vi "Read current vs temperature_3ch_2.1.1.vi"(8 "stop":bool) -> (0 "X3":cluster{"Y":dbl[], "Y":dbl[]}[](graph), 1 "Zx 4":cluster{"Y":dbl[], "Y":dbl[]}[](graph), 2 "Zx 3":cluster{"Y":dbl[], "Y":dbl[]}[](graph), 3 "Temp vs Time":cluster{"Y":dbl[], "Y":dbl[]}[](graph), 4 "i X":cluster{"Y":dbl[], "Y":dbl[]}[](graph), 5 "X 2":cluster{"Y":dbl[], "Y":dbl[]}[](graph))   [LabVIEW 2013]
uses:
  PPMS_remote/branches/sim-JL/Simulate.glb.vi
  lockin/branches/PPMS-demomode-JL/Lock-in Globles.vi
  SubVI/ITX_Global.vi
panel:
  in  "Tab Control":T1(tab)
  in  "Lockins":u16[](array[ring]) items=["Lock-in #1", "Lock-in #2", "Lock-in #3", "Lock-in #4"]
  out "OSC Configuration":T2(array[cluster])=[{"Signal Type"=enum."Sine Wave", "DC"=0.0005, "Amplitude"=0.001, "frequency"=1.346, "Phase"=0.0}, {"Signal Type"=enum."Sine Wave", "DC"=0.0, "Amplitude"=0.0, "frequency"=1.346, "Phase"=0.0}, {"Signal Type"=enum."Sine Wave", "DC"=0.0, "Amplitude"=0.0, "frequency"=1.346, "Phase"=0.0}, {"Signal Type"=enum."Sine Wave", "DC"=0.0, "Amplitude"=0.0, "frequency"=1.346, "Phase"=0.0}] {"frequency" format="%0.2p"; "Amplitude" format="%0.2p"; "DC" format="%.2p"}
  in  "milliseconds to wait":u32=1000
  in  "Comments":string="SA02610M 20130128\ncool down\n"
  out "Connected":string="I-:4\nV2+:28\nI+:1\nV1+:2\nV-:3\nV2-:5\n"
  out "i Y":cluster{"Y":dbl[], "Y":dbl[]}[](graph)
  out "i X 3":cluster{"Y":dbl[], "Y":dbl[]}[](graph)
  out "i Y 3":cluster{"Y":dbl[], "Y":dbl[]}[](graph)
  out "Y 2":cluster{"Y":dbl[], "Y":dbl[]}[](graph)
  out "Y3":cluster{"Y":dbl[], "Y":dbl[]}[](graph)
  out "Zy 3":cluster{"Y":dbl[], "Y":dbl[]}[](graph)
  out "Zy 4":cluster{"Y":dbl[], "Y":dbl[]}[](graph)
  out "i X 2":cluster{"Y":dbl[], "Y":dbl[]}[](graph)
  out "i X 4":cluster{"Y":dbl[], "Y":dbl[]}[](graph)
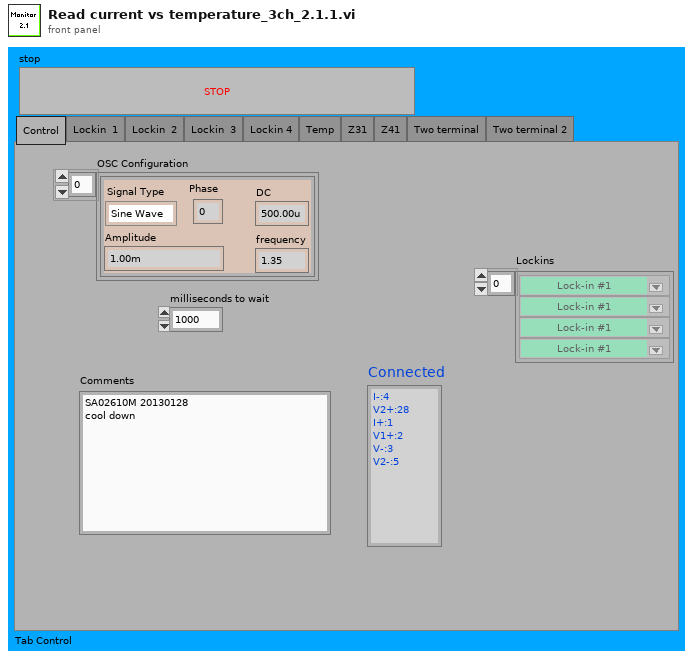
[diagram p1: front panel]
types:
  T1 = enum32{"Control", "Lockin  1", "Lockin  2", "Lockin  3", "Lockin 4", "Temp", "Z31", "Z41", "Two terminal", "Two terminal 2"}
  T2 = cluster{"Signal Type":enum16{"Sine Wave", "Triangle Wave", "Square Wave", "Sawtooth Wave"}, "DC":dbl, "Amplitude":dbl, "frequency":dbl, "Phase":dbl}[]
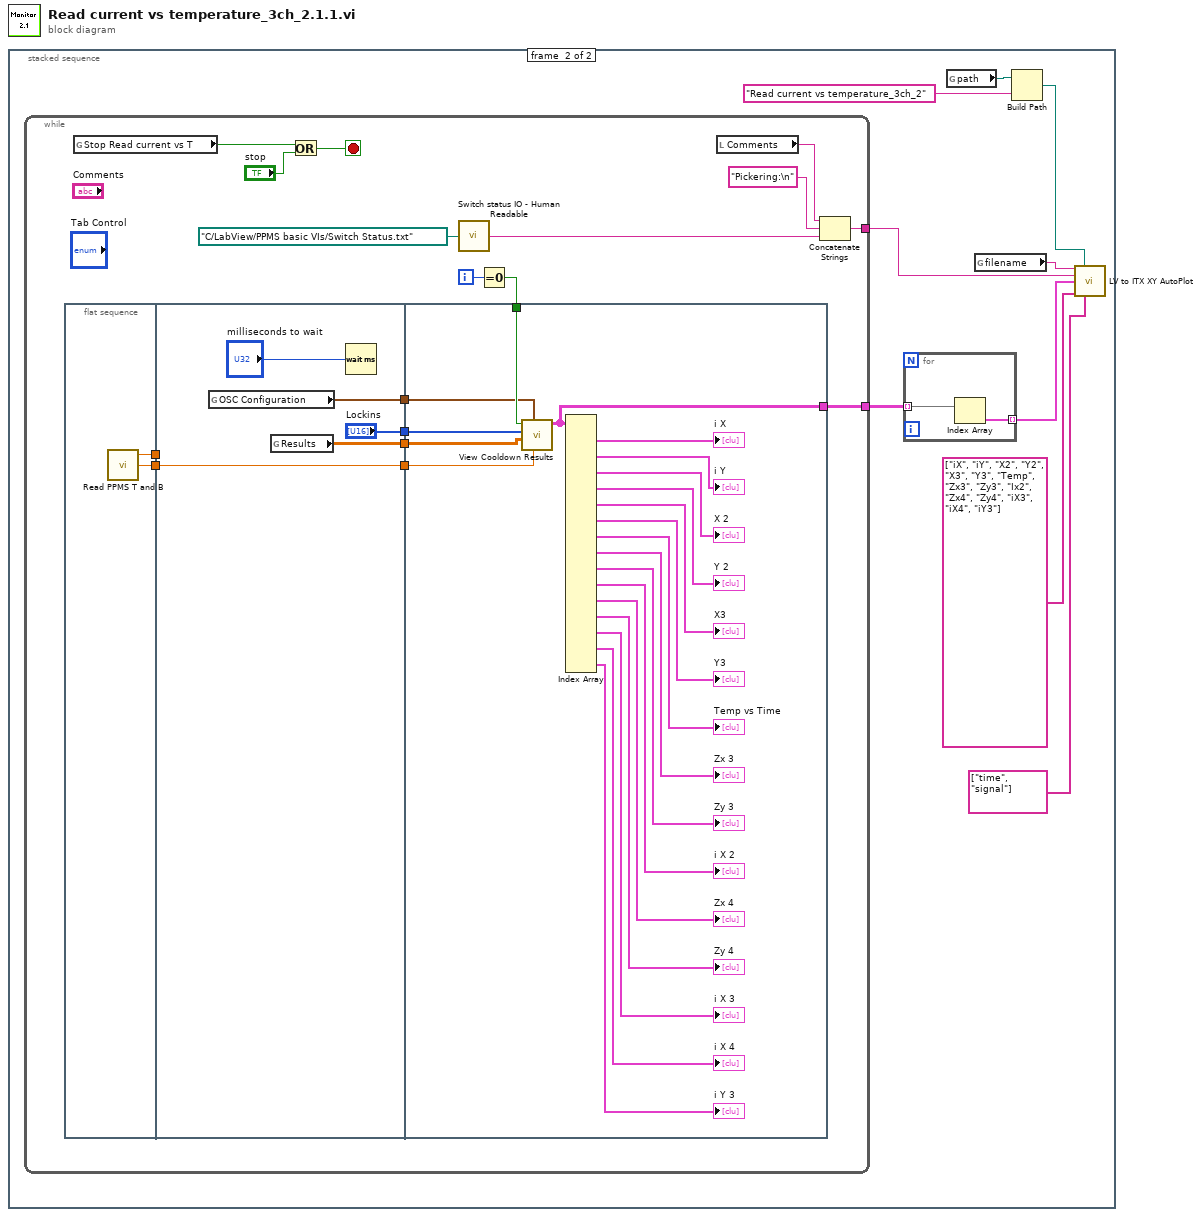
[diagram p0: block diagram]
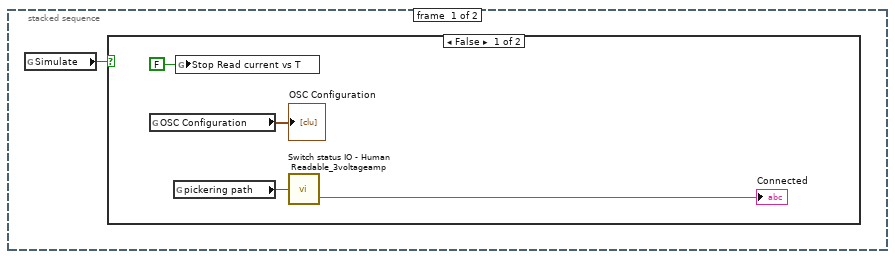
[diagram p2: hidden frame]
diagram:
  n1 = stacked-sequence {
    frame #0 {
      n2 = global read "Simulate.glb.vi" "Simulate"() -> (w1:bool)
      n3 = case shown="False" w1 {
        frame False {
          n4 = global read "Lock-in Globles.vi" "OSC Configuration"() -> (→"OSC Configuration":T2)
          n5 = global read "ITX_Global.vi" "pickering path"() -> (w2:path)
          n6 = global write "Lock-in Globles.vi" "Stop Read current vs T"(FALSE ("Stop Read current vs T")) -> ()
          n7 = call "Switch status IO - Human Readable_3voltageamp.vi"("Switch status"=w2) -> ("String"=→"Connected":string)  [unwired: 3 in]
        }
        frame True {
        }
      }
    }
    frame #1 {
      n8 = while {
        tunnel: [w25] -> w12
        tunnel: [w17] -> w6
        i -> [w31]
        stop <- w28 stop-if-true
        n9 = flat-sequence {
          tunnel: [w35] -> w32
          tunnel: [w34] -> w29
          tunnel: [w39] -> w33
          tunnel: w32 -> [w39]
          tunnel: w29 -> [_]
          tunnel: [w38] -> w20
          tunnel: ["Lockins"] -> w19
          tunnel: [w36] -> w18
          tunnel: w33 -> [w61]
          tunnel: w30 -> [w60]
          tunnel: w20 -> [w59]
          tunnel: w19 -> [w58]
          tunnel: w18 -> [w57]
          tunnel: [w52] -> w17
          frame #0 {
            n10 = call "Read PPMS T and B.vi"() -> ("Temperature"=w35:dbl, "Time"=w34:dbl)  [unwired: 3 in, 1 out]
          }
          frame #1 {
            n11 = global read "Lock-in Globles.vi" "OSC Configuration"() -> (w38:T2)
            n12 = global read "Lock-in Globles.vi" "Results"() -> (w36:dbl[][])
            n13 = Wait (ms)(milliseconds to wait="milliseconds to wait") -> ()  [unwired: 1 out]
          }
          frame #2 {
            n14 = call "View Cooldown Results.vi"("Temperature"=w61, "OSC Configuration"=w59, "Results"=w57, "Lockins"=w58, "Boolean"=w60) -> ("Array"=w52:cluster{"Y":dbl[], "Y":dbl[]}[][])  [unwired: 6 in]
            n15 = Index Array(array=w52) -> (element #1=→"i X":cluster{"Y":dbl[], "Y":dbl[]}[], element #2=→"i Y":cluster{"Y":dbl[], "Y":dbl[]}[], element #3=→"X 2":cluster{"Y":dbl[], "Y":dbl[]}[], element #4=→"Y 2":cluster{"Y":dbl[], "Y":dbl[]}[], element #5=→"X3":cluster{"Y":dbl[], "Y":dbl[]}[], element #6=→"Y3":cluster{"Y":dbl[], "Y":dbl[]}[], element #7=→"Temp vs Time":cluster{"Y":dbl[], "Y":dbl[]}[], element #8=→"Zx 3":cluster{"Y":dbl[], "Y":dbl[]}[], element #9=→"Zy 3":cluster{"Y":dbl[], "Y":dbl[]}[], element #10=→"i X 2":cluster{"Y":dbl[], "Y":dbl[]}[], element #11=→"Zx 4":cluster{"Y":dbl[], "Y":dbl[]}[], element #12=→"Zy 4":cluster{"Y":dbl[], "Y":dbl[]}[], element #13=→"i X 3":cluster{"Y":dbl[], "Y":dbl[]}[], element #14=→"i X 4":cluster{"Y":dbl[], "Y":dbl[]}[], element #15=→"i Y 3":cluster{"Y":dbl[], "Y":dbl[]}[])  [unwired: 30 in]
          }
        }
        n16 = global read "Lock-in Globles.vi" "Stop Read current vs T"() -> (w21:bool)
        n17 = Or(x=w21, y="stop") -> (x .or. y?=w28:bool)
        n18 = call "Switch status IO - Human Readable.vi"("Switch status"=path "C:/LabView/PPMS basic VIs/Switch Status.txt") -> ("String"=w22:string)
        n19 = Equal To 0?(x=w31) -> (x = 0?=w30:bool)
        n20 = local read "Comments"() -> (w24:string)
        n21 = Concatenate Strings(w24, "Pickering:\n" ("string"), w22) -> (w25:string)
      }
      n22 = for {
        tunnel: w6 -> [w16] mode=indexing
        tunnel: [w15] -> w14 mode=indexing
        n23 = Index Array(array=w16) -> (element=w15:cluster{"Y":dbl[], "Y":dbl[]})  [unwired: 1 in]
      }
      n24 = global read "ITX_Global.vi" "path"() -> (w9:path)
      n25 = global read "ITX_Global.vi" "filename"() -> (w13:string)
      n26 = Build Path(base path=w9, name or relative path="Read current vs temperature_3ch_2") -> (appended path=w8:path)
      n27 = call <userlib>:"LV to ITX XY AutoPlot.vi"("filename"=w13, "path"=w8, "Notes"=w12, "XY Array"=w14, "wavenames (.Vx, etc)"=string[] ["iX", "iY", "X2", "Y2", "X3", "Y3", "Temp", "Zx3", "Zy3", "Ix2", "Zx4", "Zy4", "iX3", "iX4", "iY3"], "X,Y Labels"=string[] ["time", "signal"]) -> ()  [unwired: 9 in, 1 out]
    }
  }
